vi "Measurement UI.vi"() -> ()   [LabVIEW 2021, in "Ripple_PMIC.lvlib"]
uses:
  Ripple_PMIC.lvlib
panel:
  in  "Tab Control":enum32{"Ripple Voltage", "Hidden Page"}(tab)
  out "OutputVoltageV/STimeGraph":waveform(dbl)(graph) caption="Ripple"
  in  "Source resource name":string caption="SOURCE DEVICE NAME"
  in  "Load resource name":string caption="LOAD DEVICE NAME"
  in  "Scope resource name":string caption="SCOPE DEVICE NAME"
  out "Source voltage":dbl caption="SOURCE VOLTAGE"
  out "Load current":dbl caption="LOAD CURRENT"
  out "RMS ripple voltage":dbl caption="RMS RIPPLE VOLTAGE"
  out "P-P ripple voltage":dbl caption="P-P RIPPLE VOLTAGE"
  out "Source current":dbl caption="SOURCE CURRENT"
  out "Load voltage":dbl caption="LOAD VOLATGE"
  out "Ripple values":dbl[](array[numeric]) caption="RIPPLE VALUES"
  out "dt":dbl caption="DT"
  out "Results":string[][](table) caption="RESULTS"
  in  "Load sense":i32(ring)=1009 caption="SENSE" items=["Local"=1008, "Remote"=1009]
  in  "Source sense":i32(ring)=1009 caption="SENSE" items=["Local"=1008, "Remote"=1009]
  in  "Aperture time":dbl=0.005 caption="APERTURE TIME" format="%#_6ps"
  in  "DUT setup time":dbl=1.0 caption="DUT SETUP TIME" format="%#_6ps"
  in  "Measurement configuration":string="Measurement settings"
  out "Status":string
  in  "Scope probe attenuation":dbl=1.0 caption="PROBE ATTENUATION"
  in  "Source configuration":string="Source configuration"
  in  "Scope configuration":string="Scope configuration"
  in  "Load configuration":string="Load configuration"
  in  "Mode of operation":T1(ring)=enum."Perform measurement" caption="MODE OF OPERATION"
  in  "Scope acquisition time":dbl=3.0 caption="ACQUISTION TIME" format="%#_6ps"
  in  "Scope sample rate":dbl=10000.0 caption="SAMPLE RATE" format="%#_6pHz"
  in  "Scope channel name":string="0" caption="CHANNEL NAME"
  in  "ScopeResourceName":refnum<k15> caption="RESOURCE NAME"
  in  "Load voltage limit range":dbl=6.0 caption="VOLTAGE LIMIT RANGE" format="%#_6pV"
  in  "Load current level":dbl=1.0 caption="CURRENT LEVEL" format="%#_6pA"
  in  "ELOADResourceName":refnum<k15> caption="RESOURCE NAME"
  in  "Source current limit":dbl=15.0 caption="CURRENT LIMIT" format="%#_6pA"
  in  "Source voltage level":dbl=10.0 caption="VOLTAGE LEVEL" format="%#_6pV"
  in  "PPSResourceName":refnum<k15> caption="RESOURCE NAME"
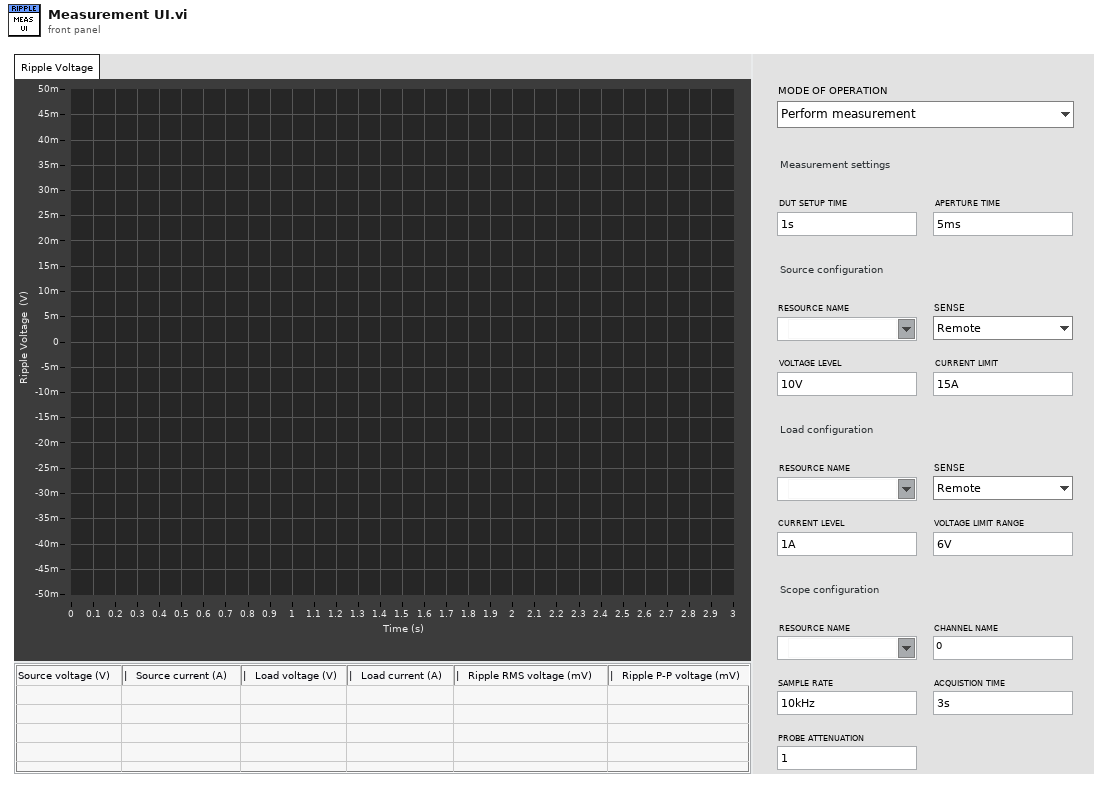
[diagram p1: front panel]
types:
  T1 = enum32{"Power on the DUT", "Perform measurement", "Power off the DUT"}
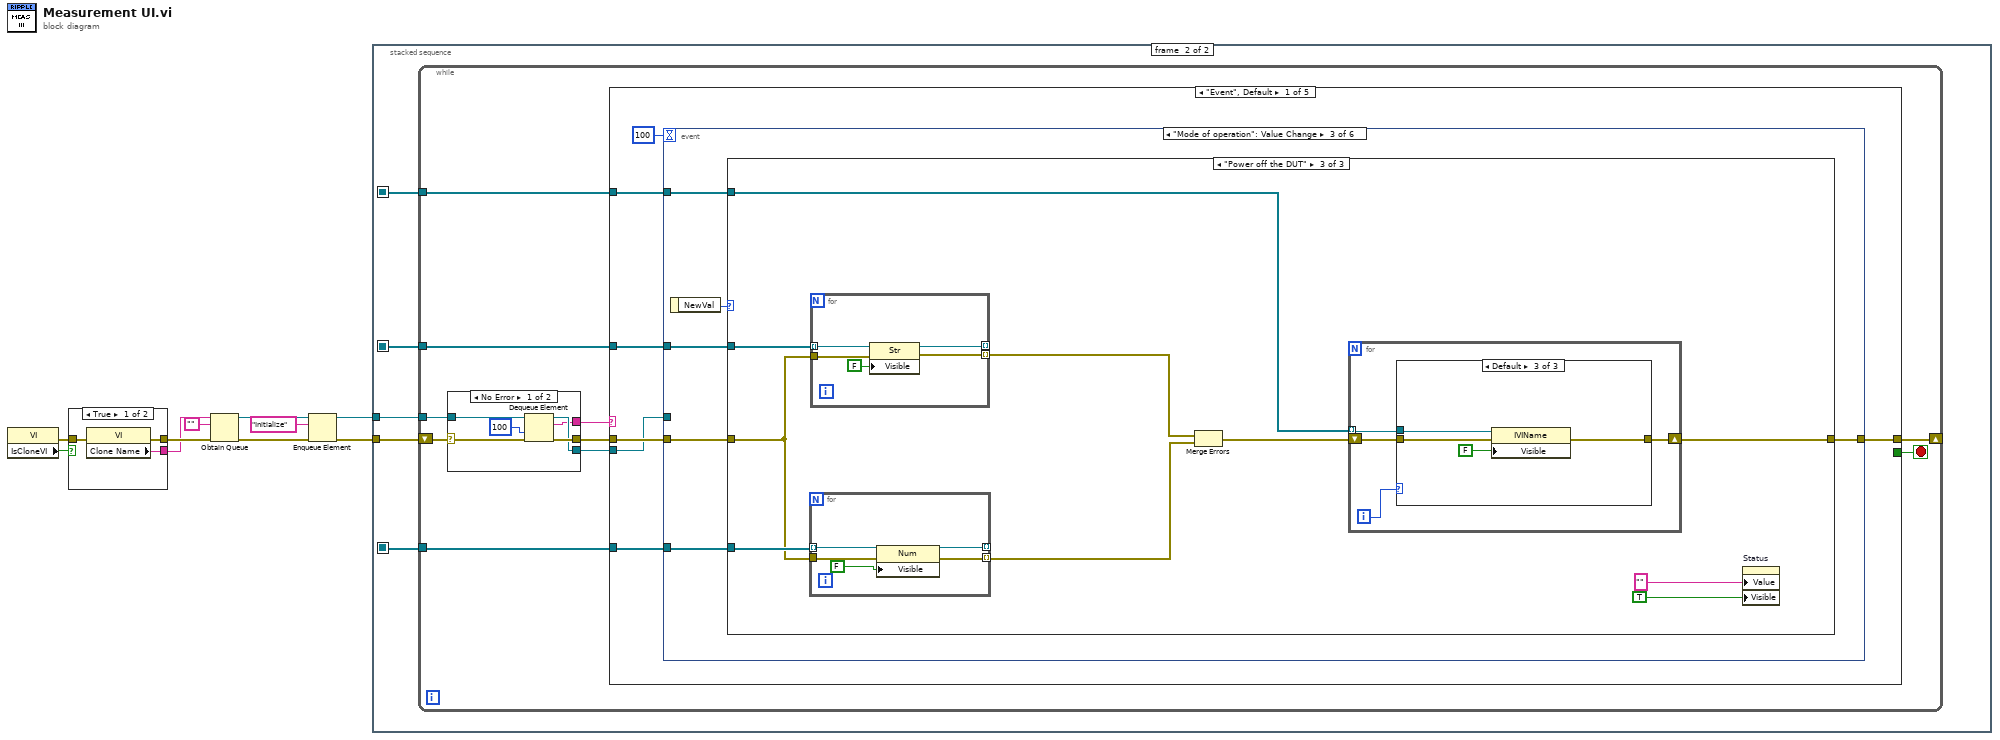
[diagram p0: block diagram]
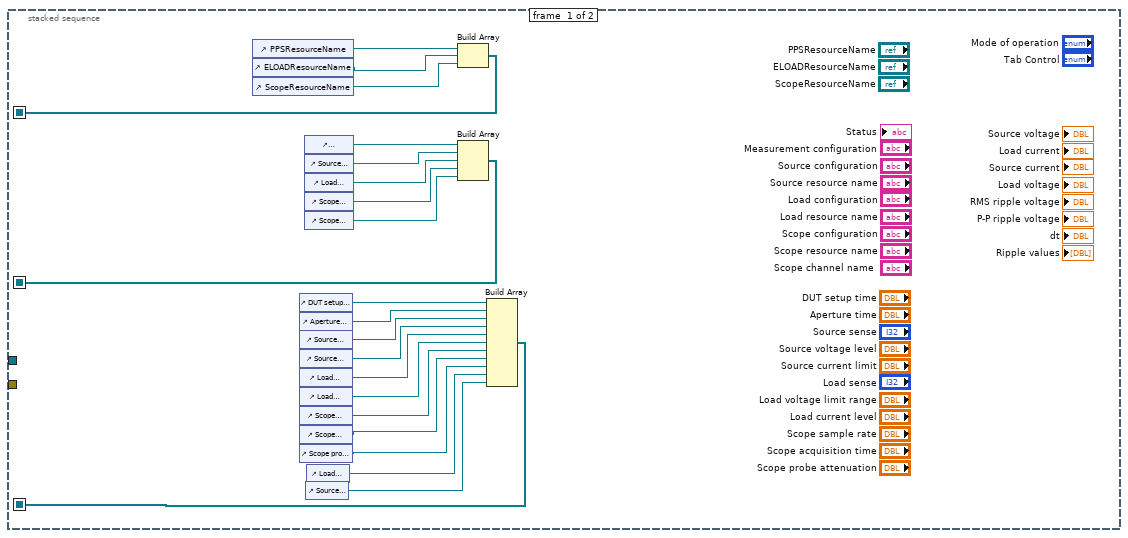
[diagram p2: hidden frame]
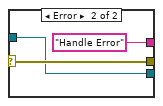
[diagram p3: hidden frame]
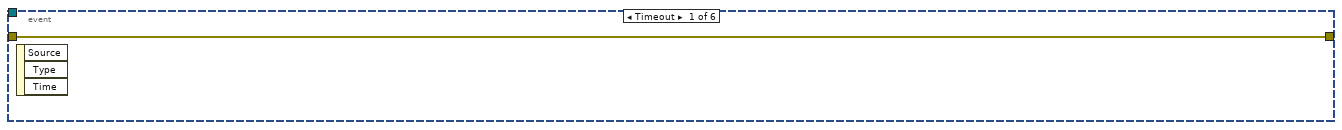
[diagram p4: hidden frame]
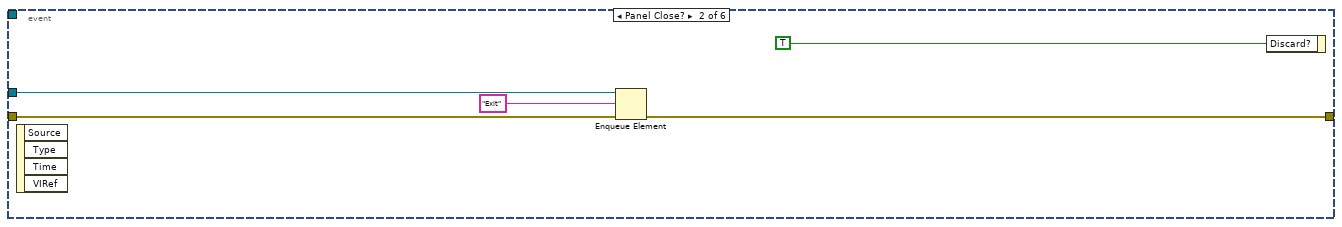
[diagram p5: hidden frame]
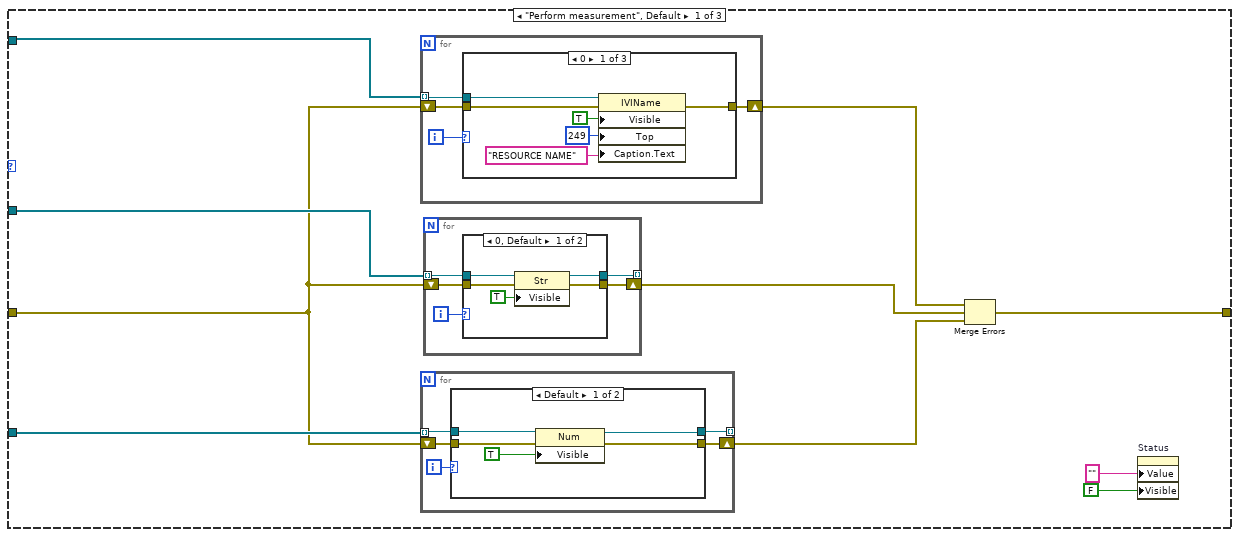
[diagram p6: hidden frame]
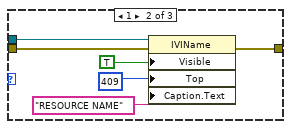
[diagram p7: hidden frame]
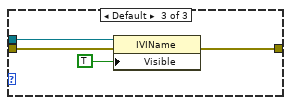
[diagram p8: hidden frame]
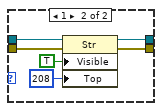
[diagram p9: hidden frame]
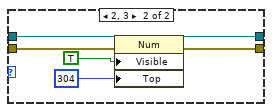
[diagram p10: hidden frame]
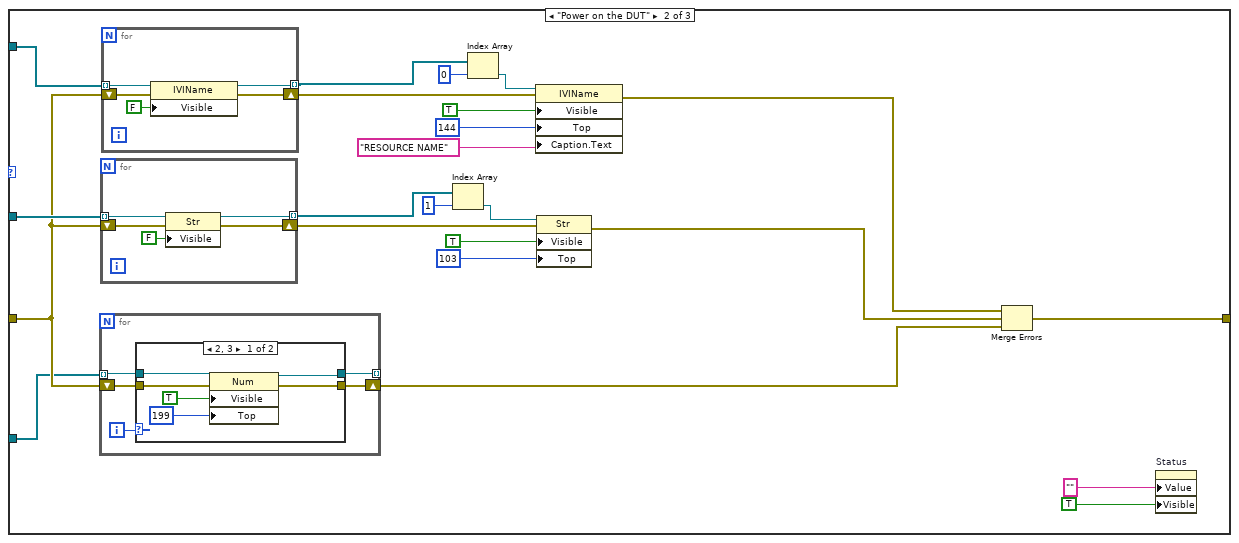
[diagram p11: hidden frame]
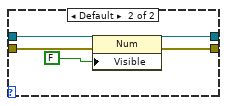
[diagram p12: hidden frame]
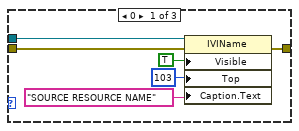
[diagram p13: hidden frame]
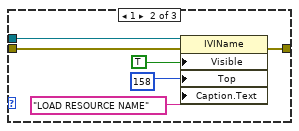
[diagram p14: hidden frame]
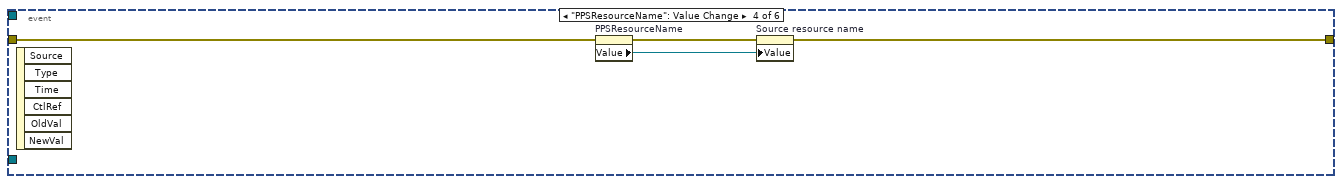
[diagram p15: hidden frame]
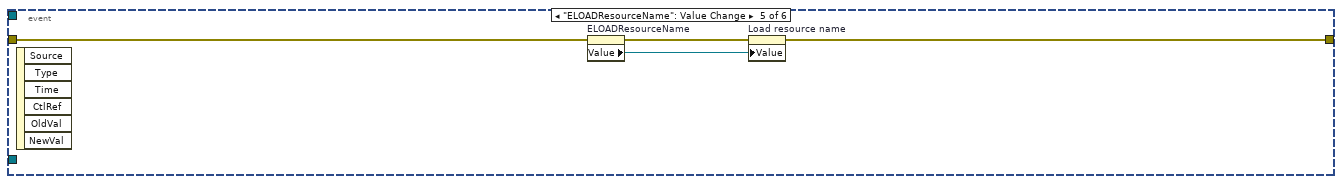
[diagram p16: hidden frame]
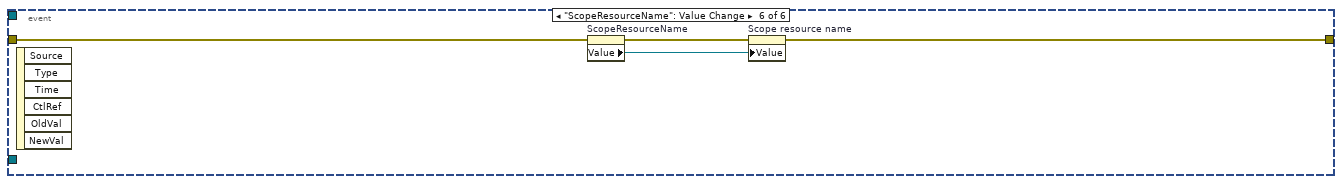
[diagram p17: hidden frame]
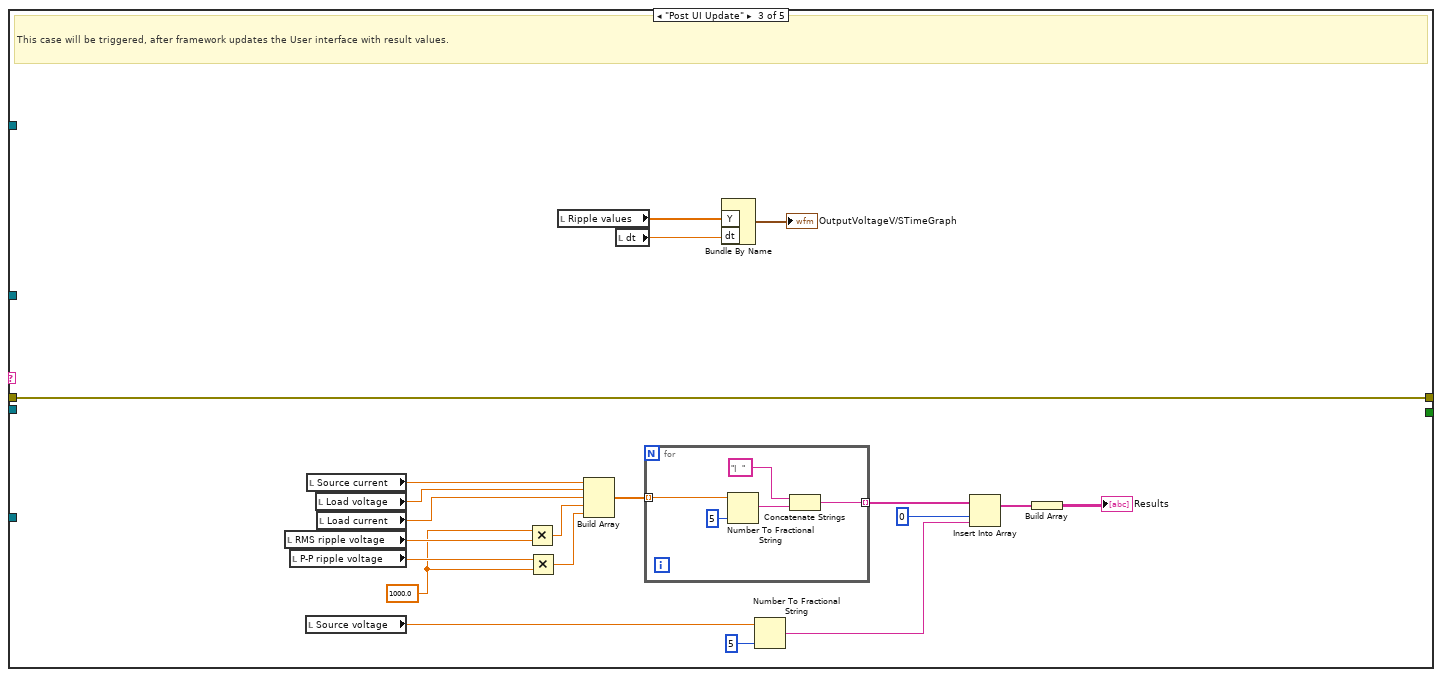
[diagram p19: hidden frame]
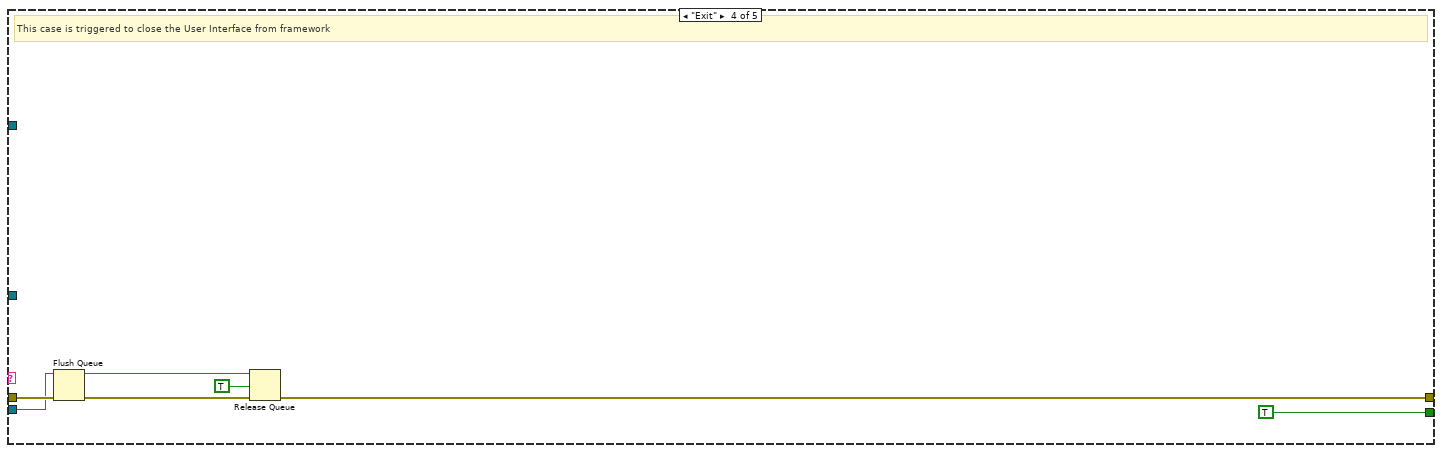
[diagram p20: hidden frame]
diagram:
  n1 = property class="VI"() -> (error out=w1:errorcluster, "IsCloneVI"=w2:bool)  [unwired: 2 in, 1 out]
  n2 = case shown="True" w2 {
    tunnel: [w13 w16] -> w10
    tunnel: [w12 w15] -> w9
    tunnel: w1 -> [w11 w14]
    frame True {
      n3 = property class="VI"(error in=w11) -> (error out=w13:errorcluster, "Clone Name"=w12:string)  [unwired: 1 in, 1 out]
    }
    frame False {
      n4 = property class="VI"(error in=w14) -> (error out=w16:errorcluster, "Name"=w15:string)  [unwired: 1 in, 1 out]
    }
  }
  n5 = Obtain Queue(name (unnamed)=w9, element data type="", error in (no error)=w10) -> (queue out=w6:refnum<queue>, error out=w8:errorcluster)  [unwired: 2 in, 1 out]
  n6 = Enqueue Element(queue=w6, element="Initialize", error in (no error)=w8) -> (queue out=w5:refnum<queue>, error out=w7:errorcluster)  [unwired: 1 in, 1 out]
  n7 = stacked-sequence {
    seq-local: [w27 _] -> [_ w39]
    seq-local: [w26 _] -> [_ w41]
    seq-local: [w25 _] -> [_ w40]
    tunnel: w7 -> [_ w43]
    tunnel: w5 -> [_ w42]
    frame #0 {
      n8 = control-ref of="PPSResourceName"() -> (w30:refnum<vi>)
      n9 = control-ref of="ELOADResourceName"() -> (w29:refnum<vi>)
      n10 = control-ref of="ScopeResourceName"() -> (w28:refnum<vi>)
      n11 = control-ref of="DUT setup time"() -> (w20:refnum<vi>)
      n12 = control-ref of="Aperture time"() -> (w19:refnum<vi>)
      n13 = control-ref of="Source voltage level"() -> (w38:refnum<vi>)
      n14 = control-ref of="Source current limit"() -> (w36:refnum<vi>)
      n15 = control-ref of="Load voltage limit range"() -> (w34:refnum<vi>)
      n16 = control-ref of="Load current level"() -> (w33:refnum<vi>)
      n17 = control-ref of="Scope sample rate"() -> (w32:refnum<vi>)
      n18 = control-ref of="Scope acquisition time"() -> (w35:refnum<vi>)
      n19 = control-ref of="Scope probe attenuation"() -> (w37:refnum<vi>)
      n20 = control-ref of="Measurement configuration"() -> (w21:refnum<vi>)
      n21 = control-ref of="Source configuration"() -> (w31:refnum<vi>)
      n22 = control-ref of="Load configuration"() -> (w24:refnum<vi>)
      n23 = control-ref of="Scope configuration"() -> (w23:refnum<vi>)
      n24 = control-ref of="Scope channel name"() -> (w22:refnum<vi>)
      n25 = control-ref of="Source sense"() -> (w17:refnum<vi>)
      n26 = control-ref of="Load sense"() -> (w18:refnum<vi>)
      n27 = Build Array(w30, w29, w28) -> (w27:refnum<vi>[])
      n28 = Build Array(w21, w31, w24, w23, w22) -> (w26:refnum<vi>[])
      n29 = Build Array(w20, w19, w38, w36, w34, w33, w32, w35, w37, w18, w17) -> (w25:refnum<vi>[])
    }
    frame #1 {
      n30 = while {
        shift-right: [w48] -> _
        shift-left: w43 -> [w53]
        tunnel: w42 -> [w51]
        tunnel: w41 -> [w46]
        tunnel: w40 -> [w45]
        tunnel: w39 -> [w44]
        stop <- w47 stop-if-true
        n31 = case shown="No Error" w53 {
          selector: w53 -> [w59 w62]
          tunnel: [w58 w62] -> w52
          tunnel: w51 -> [w57 w61]
          tunnel: [w56 w61] -> w50
          tunnel: [w55 "Handle Error"] -> w49
          frame No Error {
            n32 = Dequeue Element(queue=w57, timeout in ms (-1)=100, error in (no error)=w59) -> (queue out=w56:refnum<queue>, element=w55:string, error out=w58:errorcluster)  [unwired: 1 out]
          }
          frame Error {
          }
        }
        n33 = case shown="\"Event\", Default" w49 {
          tunnel: w52 -> [w68 w245 w253 w277 w278]
          tunnel: w50 -> [w67 _ _ w275 _]
          tunnel: [w69 w245 w253 w272 w278] -> w48
          tunnel: [_ _ _ TRUE _] -> w47
          tunnel: w46 -> [w65 _ _ _ _]
          tunnel: w45 -> [w64 _ _ _ _]
          tunnel: w44 -> [w63 _ _ _ _]
          frame "Event", Default {
            n34 = event shown="[2] \"Mode of operation\": Value Change" {
              selector: _ -> [_ _ _ _ _ _]
              dyn-events: _ -> [_ _ _ _ _ _]
              timeout: 100 -> [_ _ _ _ _ _]
              tunnel: [w70 w74 w76 w233 w237 w241] -> w69
              tunnel: w68 -> [w70 w75 w81 w235 w239 w243]
              tunnel: w67 -> [_ w73 _ _ _ _]
              tunnel: w65 -> [_ _ w79 _ _ _]
              tunnel: w64 -> [_ _ w78 _ _ _]
              tunnel: w63 -> [_ _ w77 _ _ _]
              event Timeout {
                n35 = event-data() -> ()  [unwired: 1 in, 3 out]
              }
              event Panel Close? {
                n36 = event-data() -> ()  [unwired: 1 in, 4 out]
                n37 = Enqueue Element(queue=w73, element="Exit", error in (no error)=w75) -> (error out=w74:errorcluster)  [unwired: 1 in, 2 out]
                n38 = event-data("Discard?"=TRUE) -> ()  [unwired: 1 in, 1 out]
              }
              event "Mode of operation": Value Change {
                n39 = event-data() -> ("NewVal"=w80:T1)  [unwired: 1 in]
                n40 = case shown="\"Power off the DUT\"" w80 {
                  tunnel: w81 -> [w86 w159 w200]
                  tunnel: w79 -> [w91 w166 w201]
                  tunnel: w78 -> [w90 w158 w202]
                  tunnel: w77 -> [w89 w160 w199]
                  tunnel: [w85 w148 w195] -> w76
                  frame "Perform measurement", Default {
                    n41 = for {
                      shift-right: [w93] -> w84
                      shift-left: w86 -> [w94]
                      tunnel: w89 -> [w92] mode=indexing
                      i -> [w95]
                      n42 = case shown="0" w95 {
                        tunnel: w94 -> [w98 w104 w111]
                        tunnel: [w97 w103 w109] -> w93
                        tunnel: w92 -> [w96 w102 w108]
                        frame 0 {
                          n43 = property class="IVIName"(reference=w96, error in=w98, "Visible"=TRUE, "Top"=249 ("Position:Top"), "Caption.Text"="RESOURCE NAME") -> (error out=w97:errorcluster)  [unwired: 1 out]
                        }
                        frame 1 {
                          n44 = property class="IVIName"(reference=w102, error in=w104, "Visible"=TRUE, "Top"=409 ("Position:Top"), "Caption.Text"="RESOURCE NAME") -> (error out=w103:errorcluster)  [unwired: 1 out]
                        }
                        frame Default {
                          n45 = property class="IVIName"(reference=w108, error in=w111, "Visible"=TRUE) -> (error out=w109:errorcluster)  [unwired: 1 out]
                        }
                      }
                    }
                    n46 = for {
                      tunnel: w90 -> [w132] mode=indexing
                      tunnel: [w131] -> _ mode=indexing
                      shift-right: [w129] -> w82
                      shift-left: w86 -> [w130]
                      i -> [w128]
                      n47 = case shown="Default" w128 {
                        tunnel: w132 -> [w137 w143]
                        tunnel: [w134 w141] -> w131
                        tunnel: w130 -> [w136 w140]
                        tunnel: [w135 w139] -> w129
                        frame Default {
                          n48 = property class="Num"(reference=w137, error in=w136, "Visible"=TRUE) -> (reference out=w134:refnum<vi>, error out=w135:errorcluster)
                        }
                        frame 2, 3 {
                          n49 = property class="Num"(reference=w143, error in=w140, "Visible"=TRUE, "Top"=304 ("Position:Top")) -> (reference out=w141:refnum<vi>, error out=w139:errorcluster)
                        }
                      }
                    }
                    n50 = for {
                      tunnel: w91 -> [w116] mode=indexing
                      tunnel: [w114] -> _ mode=indexing
                      shift-right: [w113] -> w83
                      shift-left: w86 -> [w115]
                      i -> [w112]
                      n51 = case shown="0, Default" w112 {
                        tunnel: w116 -> [w120 w126]
                        tunnel: w115 -> [w117 w125]
                        tunnel: [w119 w124] -> w114
                        tunnel: [w118 w123] -> w113
                        frame 0, Default {
                          n52 = property class="Str"(reference=w120, error in=w117, "Visible"=TRUE) -> (reference out=w119:refnum<vi>, error out=w118:errorcluster)
                        }
                        frame 1 {
                          n53 = property class="Str"(reference=w126, error in=w125, "Visible"=TRUE, "Top"=208 ("Position:Top")) -> (reference out=w124:refnum<vi>, error out=w123:errorcluster)
                        }
                      }
                    }
                    n54 = Merge Errors(w84, w83, w82) -> (w85:errorcluster)
                    n55 = property on="Status" class="Str"("Value"="" ("Status"), "Visible"=FALSE) -> ()  [unwired: 2 in, 2 out]
                  }
                  frame "Power on the DUT" {
                    n56 = for {
                      tunnel: w158 -> [w181] mode=indexing
                      tunnel: [w180] -> _ mode=indexing
                      shift-right: [w178] -> w144
                      shift-left: w159 -> [w179]
                      i -> [w177]
                      n57 = case shown="2, 3" w177 {
                        tunnel: w181 -> [w185 w192]
                        tunnel: [w187 w190] -> w180
                        tunnel: w179 -> [w184 w189]
                        tunnel: [w186 w188] -> w178
                        frame 2, 3 {
                          n58 = property class="Num"(reference=w185, error in=w184, "Visible"=TRUE, "Top"=199 ("Position:Top")) -> (reference out=w187:refnum<vi>, error out=w186:errorcluster)
                        }
                        frame Default {
                          n59 = property class="Num"(reference=w192, error in=w189, "Visible"=FALSE) -> (reference out=w190:refnum<vi>, error out=w188:errorcluster)
                        }
                      }
                    }
                    n60 = for {
                      tunnel: w166 -> [w175] mode=indexing
                      tunnel: [w173] -> w162 mode=indexing
                      shift-right: [w172] -> w163
                      shift-left: w159 -> [w174]
                      n61 = property class="Str"(reference=w175, error in=w174, "Visible"=FALSE) -> (reference out=w173:refnum<vi>, error out=w172:errorcluster)
                    }
                    n62 = for {
                      tunnel: w160 -> [w170] mode=indexing
                      tunnel: [w168] -> w153 mode=indexing
                      shift-right: [w167] -> w154
                      shift-left: w159 -> [w169]
                      n63 = property class="IVIName"(reference=w170, error in=w169, "Visible"=FALSE) -> (reference out=w168:refnum<vi>, error out=w167:errorcluster)
                    }
                    n64 = Index Array(array=w162, index=1) -> (element=w161:refnum<vi>)
                    n65 = Index Array(array=w153, index=0) -> (element=w155:refnum<vi>)
                    n66 = property class="IVIName"(reference=w155, error in=w154, "Visible"=TRUE, "Top"=144 ("Position:Top"), "Caption.Text"="RESOURCE NAME") -> (error out=w149:errorcluster)  [unwired: 1 out]
                    n67 = property class="Str"(reference=w161, error in=w163, "Visible"=TRUE, "Top"=103 ("Position:Top")) -> (error out=w150:errorcluster)  [unwired: 1 out]
                    n68 = Merge Errors(w149, w150, w144) -> (w148:errorcluster)
                    n69 = property on="Status" class="Str"("Value"="" ("Status"), "Visible"=TRUE) -> ()  [unwired: 2 in, 2 out]
                  }
                  frame "Power off the DUT" {
                    n70 = for {
                      tunnel: w202 -> [w232] mode=indexing
                      tunnel: [w230] -> _ mode=indexing
                      tunnel: w200 -> [w229]
                      tunnel: [w228] -> w197 mode=indexing
                      n71 = property class="Num"(reference=w232, error in=w229, "Visible"=FALSE) -> (reference out=w230:refnum<vi>, error out=w228:errorcluster)
                    }
                    n72 = for {
                      tunnel: w201 -> [w226] mode=indexing
                      tunnel: w200 -> [w225]
                      tunnel: [w224] -> _ mode=indexing
                      tunnel: [w223] -> w198 mode=indexing
                      n73 = property class="Str"(reference=w226, error in=w225, "Visible"=FALSE) -> (reference out=w224:refnum<vi>, error out=w223:errorcluster)
                    }
                    n74 = Merge Errors(w198, w197) -> (w196:errorcluster)
                    n75 = for {
                      tunnel: w199 -> [w205] mode=indexing
                      shift-right: [w203] -> w195
                      shift-left: w196 -> [w204]
                      i -> [w206]
                      n76 = case shown="Default" w206 {
                        tunnel: w205 -> [w209 w214 w222]
                        tunnel: w204 -> [w208 w215 w221]
                        tunnel: [w207 w213 w219] -> w203
                        frame 0 {
                          n77 = property class="IVIName"(reference=w209, error in=w208, "Visible"=TRUE, "Top"=103 ("Position:Top"), "Caption.Text"="SOURCE RESOURCE NAME") -> (error out=w207:errorcluster)  [unwired: 1 out]
                        }
                        frame 1 {
                          n78 = property class="IVIName"(reference=w214, error in=w215, "Visible"=TRUE, "Top"=158 ("Position:Top"), "Caption.Text"="LOAD RESOURCE NAME") -> (error out=w213:errorcluster)  [unwired: 1 out]
                        }
                        frame Default {
                          n79 = property class="IVIName"(reference=w222, error in=w221, "Visible"=FALSE) -> (error out=w219:errorcluster)  [unwired: 1 out]
                        }
                      }
                    }
                    n80 = property on="Status" class="Str"("Value"="" ("Status"), "Visible"=TRUE) -> ()  [unwired: 2 in, 2 out]
                  }
                }
              }
              event "PPSResourceName": Value Change {
                n81 = event-data() -> ()  [unwired: 1 in, 6 out]
                n82 = property on="PPSResourceName" class="IVIName"(error in=w235) -> (error out=w234:errorcluster, "Value"=w236:refnum<k15>)  [unwired: 1 in, 1 out]
                n83 = property on="Source resource name" class="Str"(error in=w234, "Value"=w236) -> (error out=w233:errorcluster)  [unwired: 1 in, 1 out]
              }
              event "ELOADResourceName": Value Change {
                n84 = event-data() -> ()  [unwired: 1 in, 6 out]
                n85 = property on="ELOADResourceName" class="IVIName"(error in=w239) -> (error out=w238:errorcluster, "Value"=w240:refnum<k15>)  [unwired: 1 in, 1 out]
                n86 = property on="Load resource name" class="Str"(error in=w238, "Value"=w240) -> (error out=w237:errorcluster)  [unwired: 1 in, 1 out]
              }
              event "ScopeResourceName": Value Change {
                n87 = event-data() -> ()  [unwired: 1 in, 6 out]
                n88 = property on="ScopeResourceName" class="IVIName"(error in=w243) -> (error out=w242:errorcluster, "Value"=w244:refnum<k15>)  [unwired: 1 in, 1 out]
                n89 = property on="Scope resource name" class="Str"(error in=w242, "Value"=w244) -> (error out=w241:errorcluster)  [unwired: 1 in, 1 out]
              }
            }
          }
          frame "Initialize" {
          }
          frame "Post UI Update" {
            w250 = 1000.0 ("x")
            # "This case will be triggered, after framework updates the User interface with result values."
            n90 = local read "RMS ripple voltage"() -> (w251:dbl)
            n91 = local read "P-P ripple voltage"() -> (w252:dbl)
            n92 = local read "Source voltage"() -> (w259:dbl)
            n93 = local read "Source current"() -> (w264:dbl)
            n94 = local read "Load voltage"() -> (w263:dbl)
            n95 = local read "Load current"() -> (w262:dbl)
            n96 = Multiply(x=w250, y=w251) -> (x*y=w249:dbl)
            n97 = Multiply(x=w252, y=w250) -> (x*y=w248:dbl)
            n98 = local read "Ripple values"() -> (w246:dbl[])
            n99 = Build Array(w264, w263, w262, w249, w248) -> (w261:dbl[])
            n100 = local read "dt"() -> (w247:dbl)
            n101 = for {
              tunnel: w261 -> [w269] mode=indexing
              tunnel: [w266] -> w258 mode=indexing
              n102 = Number To Fractional String(number=w269, precision (6)=i16 5) -> (F-format string=w268:string)  [unwired: 2 in]
              n103 = Concatenate Strings("|   " ("string"), w268) -> (w266:string)
            }
            n104 = Bundle By Name("Y"=w246, "dt"=w247) -> (→"OutputVoltageV/STimeGraph":waveform(dbl))  [unwired: 1 in]
            n105 = Number To Fractional String(number=w259, precision (6)=i16 5) -> (F-format string=w257:string)  [unwired: 2 in]
            n106 = Insert Into Array(array=w258, index=0, new element=w257) -> (w255:string[])
            n107 = Build Array(w255) -> (→"Results":string[][])
          }
          frame "Exit" {
            # "This case is triggered to close the User Interface from framework"
            n108 = Flush Queue(queue=w275, error in (no error)=w277) -> (queue out=w274:refnum<queue>, error out=w273:errorcluster)  [unwired: 1 out]
            n109 = Release Queue(queue=w274, force destroy? (F)=TRUE, error in (no error)=w273) -> (error out=w272:errorcluster)  [unwired: 2 out]
          }
          frame "Handle Error" {
          }
        }
      }
    }
  }
